vi "Measurement Logic.vi"() -> ()   [LabVIEW 2022 SP3, in "Efficiency_Class D Amplifier.lvlib"]
uses:
  Efficiency_Class D Amplifier.lvlib
  <instrlib>/niDCPower/nidcpower.llb/niDCPower Source Mode.ctl
  <instrlib>/niDCPower/nidcpower.llb/niDCPower Output Function.ctl
  <instrlib>/niDMM/nidmm.llb/niDMM Configure Measurement Digits.vi
  <instrlib>/niDMM/nidmm.llb/niDMM Function.ctl
  <instrlib>/niDMM/nidmm.llb/niDMM Resolution in Digits.ctl
  Measurement Results.ctl
  <vilib>/PDM Acquisition Toolkit/host/Classes/Tasks/PCM Output/PCM Output Task.lvclass
  C:/Program Files/National Instruments/LabVIEW 2022/vi.lib/PDM Acquisition Toolkit/host/Classes/Tasks/PCM/PCM Task.lvclass
  C:/Program Files/National Instruments/LabVIEW 2022/vi.lib/PDM Acquisition Toolkit/host/Classes/Tasks/Parent/DecoderTask.lvclass
  C:/Program Files/National Instruments/LabVIEW 2022/vi.lib/PDM Acquisition Toolkit/host/Classes/Tasks/PCM Output/PCM Output Task.lvclass
  Measurement Configuration.ctl
  shared/controls/units - snr.ctl
  shared/controls/audio controls.lvlib
  shared/controls/units - ratio.ctl
  shared/controls/weighting filter.ctl
  shared/controls/lowpass filter.ctl
  shared/controls/highpass filter.ctl
  shared/controls/digital output level units.ctl
  shared/controls/power measurement method.ctl
  <vilib>/Plug-In SDKs/Measurements/Measure Call Context/Measure Call Context.lvclass
panel:
  out "Waveform Graph 2":cluster{"x0":dbl, "dx":dbl, "magnitude":dbl[]}[](graph)
  out "Waveform Graph":waveform(dbl)[](graph)
  out "measure call context out":refnum<class "Measure Call Context.lvclass">
  in  "measure call context in":refnum<class "Measure Call Context.lvclass">
  out "measurement results":T1={"channel names"=[], "frequency (Hz)"=[], "amplitude (Vrms)"=[], "amplitude (dBFS)"=[], "phase (deg)"=[], "SNR"=[], "THD+N"=[], "THD"=[], "dynamic range (dB)"=[], "gain"=[], "SFDR (dBc)"=[], "output power (W)"=[], "power supply voltage (V)"=0.0, "power supply current (A)"=0.0, "input power (W)"=0.0, "total output power (W)"=0.0, "power loss (W)"=0.0, "efficiency (%)"=0.0, "wfm - t0"=0.0, "wfm - dt"=1.9531249997269942e-05, "wfm - data"=array[12800 elements], "fft - f0"=0.0, "fft - df"=4.000000000559116, "fft - data"=array[6400 elements]}
  in  "measurement configuration":T2={"digital serial cfg file"="", "digital channel list"="7821\\PCMo 8", "master clock channel list"="7821\\PCMo 0", "signal frequency"=1000.0, "output level"=1.0, "output level units"=enum."% FS", "output range (pk-pk)"=15.0, "load impedance"=4.0, "signal phase"=0.0, "acq sampling rate"=51200.0, "min measurement cycles"=20, "min measurement time (s)"=0.1, "min settling cycles"=0, "min settling time (s)"=0.005, "acq channel"="PXI1Slot4/ai0", "band start"=20.0, "band stop"=20000.0, "weighting filter"=enum."Linear", "lowpass filter"=enum."No filter", "highpass filter"=enum."DC", "SNR units"=enum."dB", "THD+N units"=enum."dB", "THD units"=enum."dB", "gain units"=enum."dB", "power measurement method"=enum."SMU", "power measurement resource"="PXI1Slot6/0", "power supply voltage"=14.4, "power supply current limit"=1.2, "sense resistor (Ohms)"=0.01} {"acq sampling rate" format="%#_6p"}
  out "error out":errorcluster
  in  "error in":errorcluster
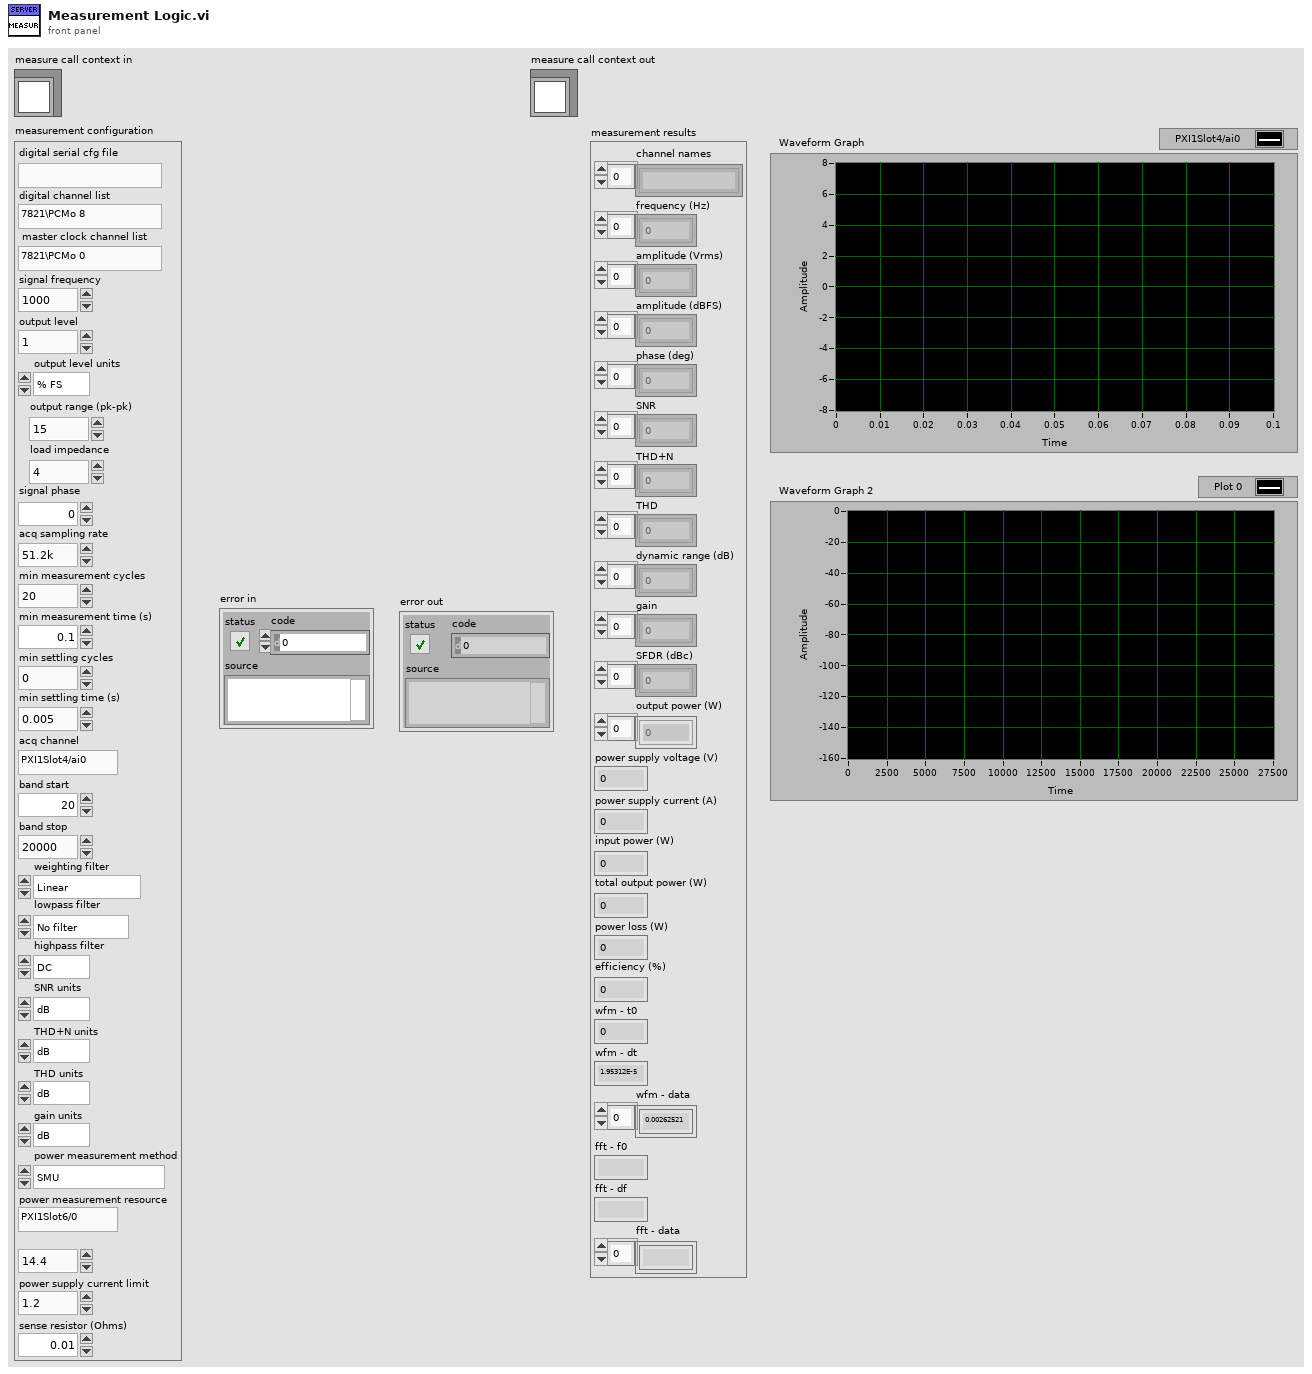
[diagram p1: front panel]
types:
  T1 = typedef "Efficiency_Class D Amplifier.lvlib/Measurement Results.ctl" = cluster{"channel names":string[], "frequency (Hz)":dbl[], "amplitude (Vrms)":dbl[], "amplitude (dBFS)":dbl[], "phase (deg)":dbl[], "SNR":dbl[], "THD+N":dbl[], "THD":dbl[], "dynamic range (dB)":dbl[], "gain":dbl[], "SFDR (dBc)":dbl[], "output power (W)":dbl[], "power supply voltage (V)":dbl, "power supply current (A)":dbl, "input power (W)":dbl, "total output power (W)":dbl, "power loss (W)":dbl, "efficiency (%)":dbl, "wfm - t0":dbl, "wfm - dt":dbl, "wfm - data":dbl[], "fft - f0":dbl, "fft - df":dbl, "fft - data":dbl[]}
  T2 = typedef "Efficiency_Class D Amplifier.lvlib/Measurement Configuration.ctl" = cluster{"digital serial cfg file":string, "digital channel list":string, "master clock channel list":string, "signal frequency":dbl, "output level":dbl, "output level units":T3, "output range (pk-pk)":dbl, "load impedance":dbl, "signal phase":dbl, "acq sampling rate":dbl, "min measurement cycles":u32, "min measurement time (s)":dbl, "min settling cycles":u32, "min settling time (s)":dbl, "acq channel":string, "band start":dbl, "band stop":dbl, "weighting filter":T4, "lowpass filter":T5, "highpass filter":T6, "SNR units":T7, "THD+N units":T8, "THD units":T8, "gain units":T8, "power measurement method":T9, "power measurement resource":string, "power supply voltage":dbl, "power supply current limit":dbl, "sense resistor (Ohms)":dbl}
  T3 = typedef "audio controls.lvlib/digital output level units.ctl" = enum32{"% FS", "dBFS", "V"}
  T4 = typedef "weighting filter.ctl" = enum32{"Linear", "A-weighting", "B-weighting", "C-weighting"}
  T5 = typedef "lowpass filter.ctl" = enum32{"No filter", "AES17 20kHz", "AES17 40kHz"}
  T6 = typedef "highpass filter.ctl" = enum32{"DC", "AC"}
  T7 = typedef "audio controls.lvlib/units - snr.ctl" = enum32{"dB", "x/y"}
  T8 = typedef "audio controls.lvlib/units - ratio.ctl" = enum32{"dB", "%", "x/y"}
  T9 = typedef "power measurement method.ctl" = enum32{"SMU", "DMM"}
  T10 = typedef "niDMM Function.ctl" = enum16{"DC Volts", "AC Volts", "DC Current", "AC Current", "2-wire Resistance", "4-wire Resistance", "Diode", "Frequency", "Period", "AC Volts DC Coupled", "Capacitance", "Inductance", "Temperature"}
  T11 = typedef "niDCPower Output Function.ctl" = i32
  T12 = typedef "niDCPower Source Mode.ctl" = i32
  T13 = typedef "niDMM Resolution in Digits.ctl" = dbl
  T14 = typedef "single tone measurement settings (HW).ctl" = cluster{"digital channel list":string, "frame clock rate":dbl, "number of channels":u32, "channel length":u32, "bit depth":u32, "data justification":T15, "endianness":T16, "bit clock edge sync":T17, "frame sync edge for channel 0":T17, "channel 0 offset":u32, "master clock channel list":string, "master clock rate":dbl, "enable dither":bool, "logic level":T18, "signal frequency":dbl, "output level":dbl, "output level units":T3, "output range (pk-pk)":dbl, "load impedance":dbl, "signal phase":dbl, "acq sampling rate":dbl, "min measurement cycles":u32, "min measurement time (s)":dbl, "min settling cycles":u32, "min settling time (s)":dbl, "acq channel":string, "band start":dbl, "band stop":dbl, "weighting filter":T4, "highpass filter":T6, "lowpass filter":T5, "SNR units":T7, "THD+N units":T8, "THD units":T8, "gain units":T8}
  T15 = typedef "data justification.ctl" = enum32{"Left Justified", "Right Justified"}
  T16 = typedef "endianness.ctl" = enum32{"MSB First", "LSB First"}
  T17 = typedef "digital edge.ctl" = enum32{"Rising", "Falling"}
  T18 = typedef "logic level.ctl" = enum32{"3.3 V", "1.8 V", "1.2 V"}
  T19 = typedef "audio controls.lvlib/single tone audio measurements.ctl" = cluster{"channel":string, "frequency (Hz)":dbl, "amplitude (Vrms)":dbl, "amplitude (dBFS)":dbl, "phase (deg)":dbl, "SNR":dbl, "THD+N":dbl, "THD":dbl, "dynamic range (dB)":dbl, "gain":dbl, "SFDR (dBc)":dbl}
  T20 = typedef "PCM tasks.ctl" = cluster{"PCM output task":T21, "PCM output task-clock":T21}
  T21 = typedef "PDM Acquisition Class Library.lvlib/PCM Output Task.lvclass/PCM Output Task DVR.ctl" = refnum<data-value>
  T22 = typedef "audio controls.lvlib/single tone audio measurements (N chan).ctl" = cluster{"channel names":string[], "frequency (Hz)":dbl[], "amplitude (Vrms)":dbl[], "amplitude (dBFS)":dbl[], "phase (deg)":dbl[], "SNR":dbl[], "THD+N":dbl[], "THD":dbl[], "dynamic range (dB)":dbl[], "gain":dbl[], "SFDR (dBc)":dbl[]}
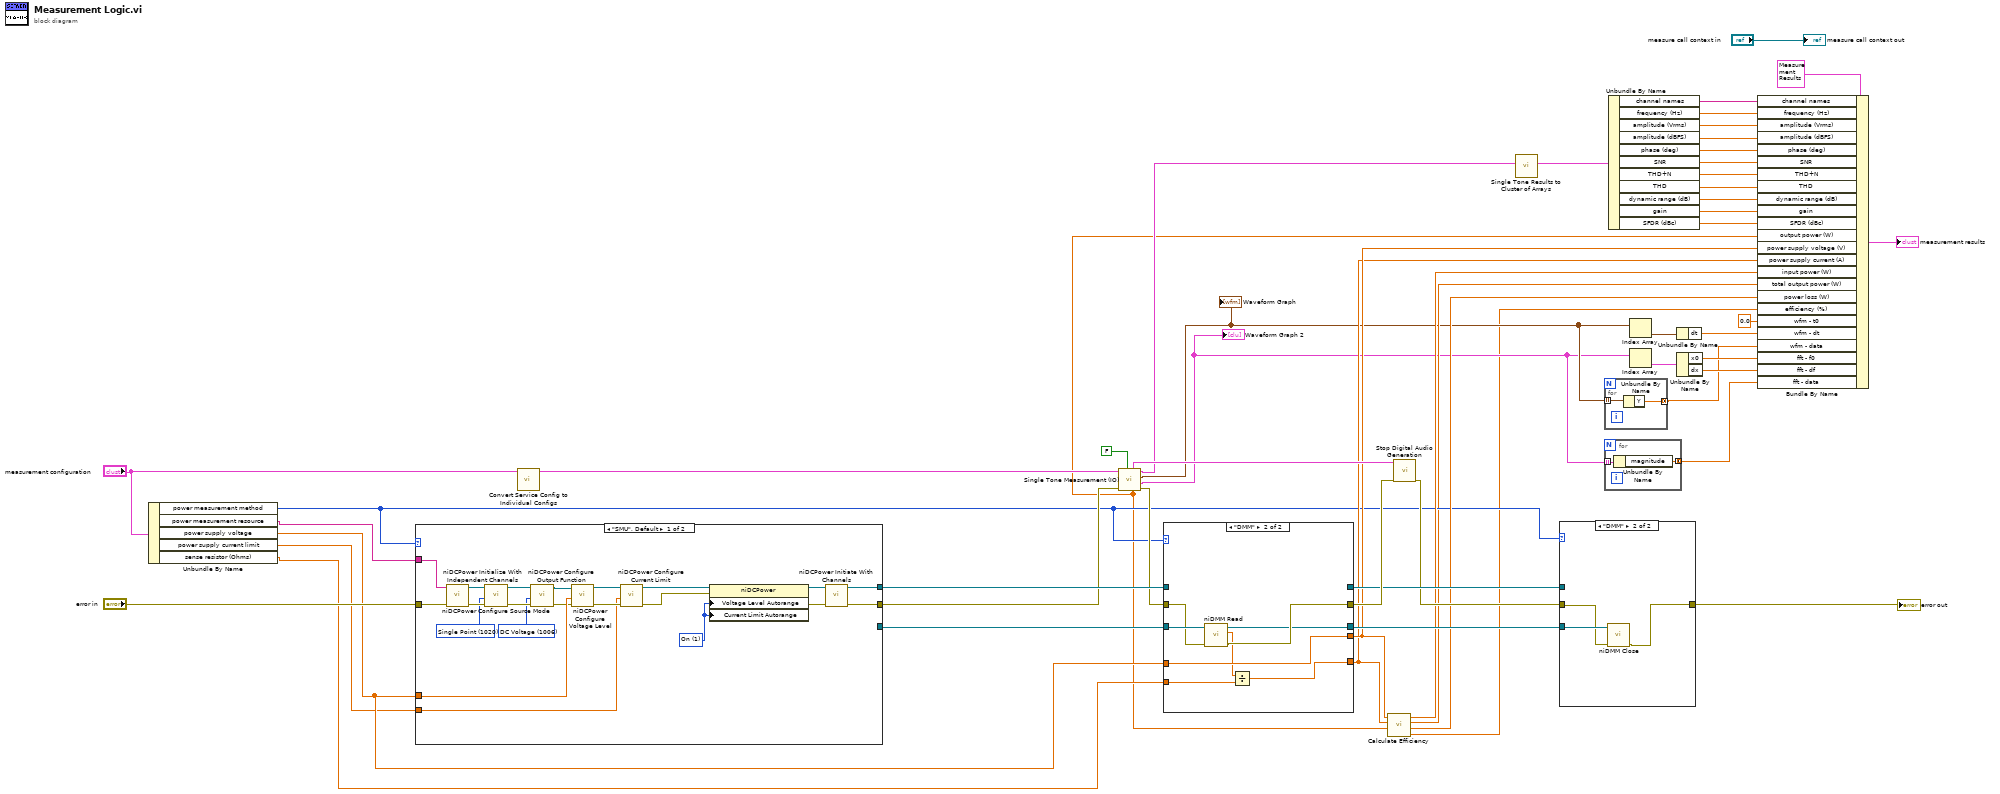
[diagram p0: block diagram]
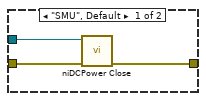
[diagram p2: hidden frame]
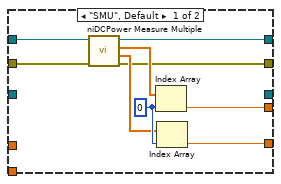
[diagram p3: hidden frame]
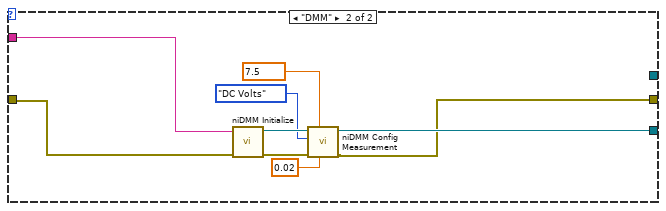
[diagram p4: hidden frame]
diagram:
  n1 = Unbundle By Name("measurement configuration") -> ("power measurement method"=w31:T9, "power measurement resource"=w30:string, "power supply voltage"=w29:dbl, "power supply current limit"=w28:dbl, "sense resistor (Ohms)"=w27:dbl)
  n2 = case shown="\"SMU\", Default" w31 {
    tunnel: w29 -> [w71 _]
    tunnel: w28 -> [w70 _]
    tunnel: [w56 _] -> w51
    tunnel: [w55 w78] -> w49
    tunnel: "error in" -> [w54 w82]
    tunnel: [_ w79] -> w42
    tunnel: w30 -> [w53 w74]
    frame "SMU", Default {
      w57 = 1 items=["Off", "On"] ("Source:DC Voltage:Current Limit Autorange")
      w58 = T11 1006 items=["DC Voltage"=1006, "DC Current"=1007, "Pulse Voltage"=1049, "Pulse Current"=1050] ("output function")
      w65 = T12 1020 items=["Single Point"=1020, "Sequence"=1021] ("source mode")
      n3 = call <instrlib>:"niDCPower Initialize With Independent Channels.vi"("error in (no error)"=w54, "resource name"=w53) -> ("error out"=w69:errorcluster, "instrument handle out"=w68:refnum<k15>)  [unwired: 8 in]
      n4 = call <instrlib>:"niDCPower Configure Source Mode.vi"("error in (no error)"=w69, "source mode"=w65, "instrument handle"=w68) -> ("error out"=w67:errorcluster, "instrument handle out"=w66:refnum<k15>)  [unwired: 7 out]
      n5 = call <instrlib>:"niDCPower Configure Output Function.vi"("error in (no error)"=w67, "output function"=w58, "instrument handle"=w66) -> ("error out"=w59:errorcluster, "instrument handle out"=w60:refnum<k15>)  [unwired: 1 in, 6 out]
      n6 = call <instrlib>:"niDCPower Configure Voltage Level.vi"("error in (no error)"=w59, "voltage level"=w71, "instrument handle"=w60) -> ("error out"=w72:errorcluster, "instrument handle out"=w73:refnum<k15>)  [unwired: 1 in, 6 out]
      n7 = call <instrlib>:"niDCPower Configure Current Limit.vi"("error in (no error)"=w72, "current limit"=w70, "instrument handle"=w73) -> ("error out"=w61:errorcluster, "instrument handle out"=w64:refnum<k15>)  [unwired: 2 in, 5 out]
      n8 = property class="niDCPower"(reference=w64, error in=w61, "Voltage Level Autorange"=w57, "Current Limit Autorange"=w57) -> (reference out=w63:refnum<k15>, error out=w62:errorcluster)
      n9 = call <instrlib>:"niDCPower Initiate With Channels.vi"("error in (no error)"=w62, "instrument handle"=w63) -> ("error out"=w55:errorcluster, "instrument handle out"=w56:refnum<k15>)  [unwired: 8 in]
    }
    frame "DMM" {
      w76 = T13 7.5 items=["3 1/2"=3.5, "4 1/2"=4.5, "5 1/2"=5.5, "6 1/2"=6.5, "7 1/2"=7.5] ("Resolution in Digits")
      n10 = call <instrlib>:"niDMM Initialize.vi"("error in (no error)"=w82, "Instrument Descriptor"=w74) -> ("error out"=w81:errorcluster, "instrument handle out"=w80:refnum<k15>)  [unwired: 8 in]
      n11 = call-poly <instrlib>:"niDMM Config Measurement.vi"("Range"=0.02, "Resolution in Digits"=w76, "error in (no error)"=w81, "Function"=niDMM_Function."DC Volts", "instrument handle"=w80) -> ("error out"=w78:errorcluster, "instrument handle out"=w79:refnum<k15>)  [unwired: 5 in]
    }
  }
  n12 = call "Convert Service Config to Individual Configs.vi"("measurement configuration"="measurement configuration") -> ("audio meas config"=w43:T14)  [unwired: 9 in, 1 out]
  n13 = call "Single Tone Measurement (IO).vi"("stop generation"=FALSE, "error in (no error)"=w49, "measurement configuration"=w43) -> ("error out"=w46:errorcluster, "spectra"=w17:cluster{"x0":dbl, "dx":dbl, "magnitude":dbl[]}[], "waveforms"=w19:waveform(dbl)[], "results"=w24:T19[], "output power"=w2:dbl[], "PCM tasks"=w44:T20)  [unwired: 3 in]
  "Waveform Graph" <- w19
  "Waveform Graph 2" <- w17
  n14 = case shown="\"DMM\"" w31 {
    tunnel: w51 -> [w91 _]
    tunnel: [w90 _] -> w41
    tunnel: [w89 w96] -> w37
    tunnel: [w88 w93] -> w36
    tunnel: [w84 w97] -> w47
    tunnel: w46 -> [w83 w98]
    tunnel: w42 -> [_ w99]
    tunnel: w27 -> [_ w94]
    tunnel: w29 -> [_ w96]
    tunnel: [_ w92] -> w39
    frame "SMU", Default {
      w87 = 0 ("index")
      n15 = call <instrlib>:"niDCPower Measure Multiple.vi"("error in (no error)"=w83, "instrument handle"=w91) -> ("error out"=w84:errorcluster, "current measurements"=w85:dbl[], "voltage measurements"=w86:dbl[], "instrument handle out"=w90:refnum<k15>)  [unwired: 6 in]
      n16 = Index Array(array=w86, index=w87) -> (element=w89:dbl)
      n17 = Index Array(array=w85, index=w87) -> (element=w88:dbl)
    }
    frame "DMM" {
      n18 = call <instrlib>:"niDMM Read.vi"("error in (no error)"=w98, "instrument handle"=w99) -> ("error out"=w97:errorcluster, "Measurement"=w95:dbl, "instrument handle out"=w92:refnum<k15>)  [unwired: 7 in]
      n19 = Divide(x=w95, y=w94) -> (x/y=w93:dbl)
    }
  }
  n20 = call "Calculate Efficiency.vi"("output power per channel"=w2, "power supply current"=w36, "power supply voltage"=w37) -> ("efficiency"=w1:dbl, "power loss"=w34:dbl, "total output power"=w25:dbl, "input power"=w35:dbl)  [unwired: 5 in]
  n21 = call "Stop Digital Audio Generation.vi"("error in (no error)"=w47, "PCM tasks"=w44) -> ("error out"=w40:errorcluster)  [unwired: 9 in]
  n22 = call "Single Tone Results to Cluster of Arrays.vi"("results"=w24) -> ("results (N chan)"=w15:T22)  [unwired: 10 in]
  n23 = case shown="\"DMM\"" w31 {
    tunnel: [w102 w103] -> w50
    tunnel: w41 -> [w101 _]
    tunnel: w40 -> [w100 w104]
    tunnel: w39 -> [_ w105]
    frame "SMU", Default {
      n24 = call <instrlib>:"niDCPower Close.vi"("error in (no error)"=w100, "instrument handle"=w101) -> ("error out"=w102:errorcluster)  [unwired: 9 out]
    }
    frame "DMM" {
      n25 = call <instrlib>:"niDMM Close.vi"("error in (no error)"=w104, "instrument handle"=w105) -> ("error out"=w103:errorcluster)  [unwired: 9 in]
    }
  }
  "error out" <- w50
  n26 = for {
    tunnel: w19 -> [w107] mode=indexing
    tunnel: [w106] -> w18 mode=concatenating
    n27 = Unbundle By Name(w107) -> ("Y"=w106:dbl[])
  }
  n28 = for {
    tunnel: w17 -> [w109] mode=indexing
    tunnel: [w108] -> w16 mode=concatenating
    n29 = Unbundle By Name(w109) -> ("magnitude"=w108:dbl[])
  }
  n30 = Unbundle By Name(w15) -> ("channel names"=w13:string[], "frequency (Hz)"=w12:dbl[], "amplitude (Vrms)"=w11:dbl[], "amplitude (dBFS)"=w10:dbl[], "phase (deg)"=w9:dbl[], "SNR"=w8:dbl[], "THD+N"=w7:dbl[], "THD"=w6:dbl[], "dynamic range (dB)"=w5:dbl[], "gain"=w4:dbl[], "SFDR (dBc)"=w3:dbl[])
  n31 = Index Array(array=w19) -> (element=w22:waveform(dbl))  [unwired: 1 in]
  n32 = Index Array(array=w17) -> (element=w23:cluster{"x0":dbl, "dx":dbl, "magnitude":dbl[]})  [unwired: 1 in]
  n33 = Unbundle By Name(w22) -> ("dt"=w33:dbl)
  n34 = Unbundle By Name(w23) -> ("x0"=w21:dbl, "dx"=w20:dbl)
  n35 = Bundle By Name(cluster=T1 {"channel names"=[], "frequency (Hz)"=[], "amplitude (Vrms)"=[], "amplitude (dBFS)"=[], "phase (deg)"=[], "SNR"=[], "THD+N"=[], "THD"=[], "dynamic range (dB)"=[], "gain"=[], "SFDR (dBc)"=[], "output power (W)"=[], "power supply voltage (V)"=0.0, "power supply current (A)"=0.0, "input power (W)"=0.0, "total output power (W)"=0.0, "power loss (W)"=0.0, "efficiency (%)"=0.0, "wfm - t0"=0.0, "wfm - dt"=1.9531249997269942e-05, "wfm - data"=array[12800 elements], "fft - f0"=0.0, "fft - df"=4.000000000559116, "fft - data"=array[6400 elements]} ("measurement results"), "channel names"=w13, "frequency (Hz)"=w12, "amplitude (Vrms)"=w11, "amplitude (dBFS)"=w10, "phase (deg)"=w9, "SNR"=w8, "THD+N"=w7, "THD"=w6, "dynamic range (dB)"=w5, "gain"=w4, "SFDR (dBc)"=w3, "output power (W)"=w2, "power supply voltage (V)"=w37, "power supply current (A)"=w36, "input power (W)"=w35, "total output power (W)"=w25, "power loss (W)"=w34, "efficiency (%)"=w1, "wfm - t0"=0.0, "wfm - dt"=w33, "wfm - data"=w18, "fft - f0"=w21, "fft - df"=w20, "fft - data"=w16) -> (→"measurement results":T1)
  "measure call context out" <- "measure call context in"
